vi "Initialize.vi"(8 "error in (no error)":errorcluster, 10 "ActivationHandler in":refnum<class "ActivationHandler.lvclass">) -> (0 "error out":errorcluster, 2 "ActivationHandler out":refnum<class "ActivationHandler.lvclass">, 3 "ToastService out":refnum<class "ToastService.lvclass">)   [LabVIEW 2026, in "ToastNotification.lvlib" / "ToastService.lvclass"]
doc: "Initialize a new ToastService and the supplied ActivationHandler. Call WasCurrentProcessToastActivated for native toolkit initialization, call the handler Initialize hook, then store the native reference and initialized handler in the service. Return the initialized handler so the caller can borrow resources created by its hook. Call Register For Events separately before Show. Skip on incoming error, returning a default service and the unchanged input handler. Partial initialization has no rollback guarantee."
uses:
  ToastService.lvclass
  ActivationHandler/ActivationHandler.lvclass
  ToastService.lvclass/ToastService.ctl
  Write ActivationHandler.vi
  Write reference.vi
  C:/Users/loicw/Documents/LabVIEW/ToastNotifications/Sources/bins/Microsoft.Toolkit.Uwp.Notifications.dll
  bins/Microsoft.Toolkit.Uwp.Notifications.dll
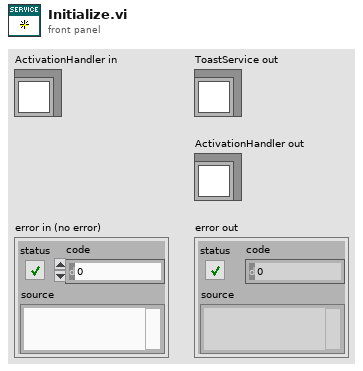
[diagram p1: front panel]
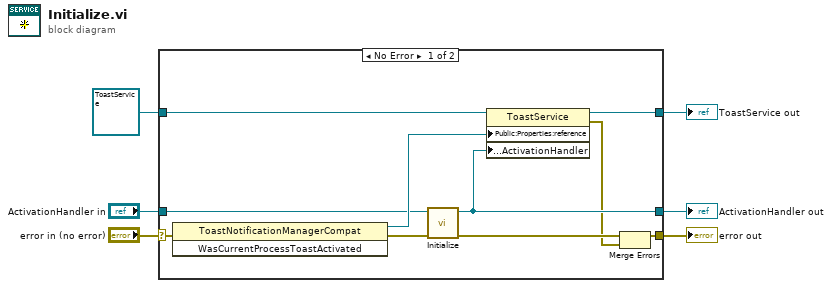
[diagram p0: block diagram]
diagram:
  n1 = case shown="No Error" "error in (no error)" {
    selector: "error in (no error)" -> [w15 w19]
    tunnel: refnum<class "ToastService.lvclass"> refnum -> [w16 w18]
    tunnel: [w14 w18] -> w4
    tunnel: [w9 w19] -> w3
    tunnel: "ActivationHandler in" -> [w11 w17]
    tunnel: [w10 w17] -> w1
    frame No Error {
      n2 = invoke class="ToastNotificationManagerCompat" method="WasCurrentProcessToastActivated"(error in=w15) -> (reference out=w13:refnum<k24>, error out=w12:errorcluster)  [unwired: 2 in, 1 out]
      n3 = call-dynamic "Initialize.vi"("error in (no error)"=w12, "ActivationHandler in"=w11) -> ("error out"=w8:errorcluster, "ActivationHandler out"=w10:refnum<class "ActivationHandler.lvclass">)  [unwired: 8 in]
      n4 = property class="ToastService"(reference=w16, "Public:Properties:reference"=w13, "Public:Properties:ActivationHandler"=w10) -> (reference out=w14:refnum<class "ToastService.lvclass">, error out=w7:errorcluster)  [unwired: 1 in]
      n5 = Merge Errors(w8, w7) -> (w9:errorcluster)
    }
    frame Error {
    }
  }
  "ToastService out" <- w4
  "error out" <- w3
  "ActivationHandler out" <- w1
